vi "lvgit push.vi"(8 "error in":errorcluster, 11 "path":path) -> (0 "error out":errorcluster)   [LabVIEW 2017]
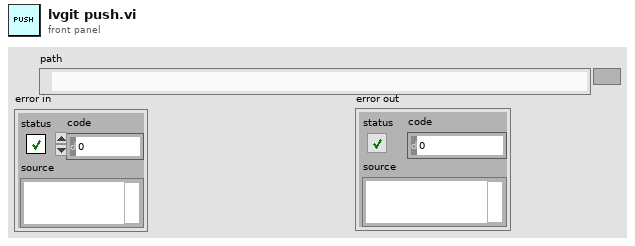
[diagram p1: front panel]
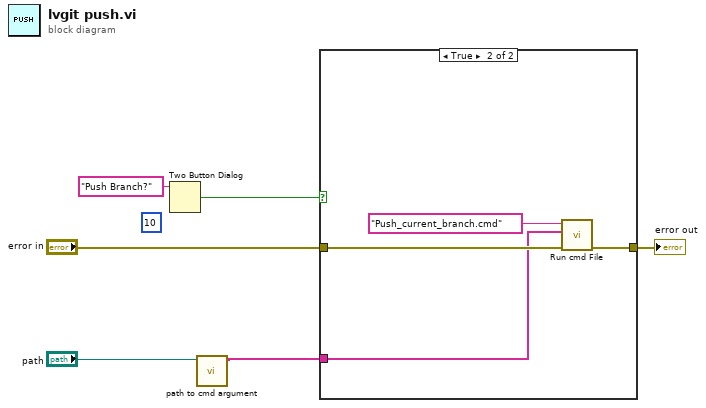
[diagram p0: block diagram]
diagram:
  (unwired) 10 ("F Timeout(-1 s)")
  n1 = Two Button Dialog(message="Push Branch?") -> (T button?=w5:bool)  [unwired: 2 in]
  n2 = call "path to cmd argument.vi"("path"="path") -> ("Array"=w1:string[])  [unwired: 10 in]
  n3 = case shown="True" w5 {
    tunnel: "error in" -> [w7 w11]
    tunnel: [w7 w10] -> w4
    tunnel: w1 -> [_ w8]
    frame False {
    }
    frame True {
      n4 = call "Run cmd File.vi"("Error in"=w11, "args"=w8, "name or relative path"="Push_current_branch.cmd") -> ("Error out"=w10:errorcluster)  [unwired: 6 in, 2 out]
    }
  }
  "error out" <- w4
